vi "Get Main Menu.vi"(8 "error in":errorcluster) -> (0 "error out":errorcluster, 3 "Main Menu":T1)   [LabVIEW 2026]
doc: "Returns the ATM Main Menu as data: for each of the six function buttons the label shown beside it and the state the main state machine runs when it is pressed. Left side: Fast Cash $100, Balance Inquiry, Return Card and Terminate. Right side: Deposit, Withdraw, Fast Cash $50. To change a label or to move an item to another button, edit the Main Menu constant; the main state machine needs no change for that. An item with a NEW action also needs a new item in ATM States.ctl and a case for it in the main state machine - an action without a case of its own runs the \"None\", Default case and does nothing.\n\nError behaviour: error in is passed to error out unchanged; the menu is returned in every case."
uses:
  Controls/ATM Menu.ctl
  Controls/ATM Menu Side.ctl
  Controls/ATM Menu Item.ctl
  Controls/ATM States.ctl
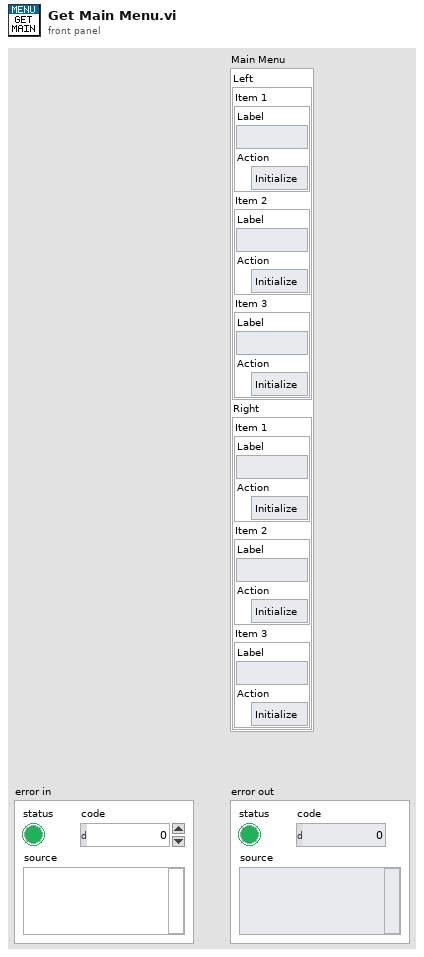
[diagram p1: front panel]
types:
  T1 = typedef "ATM Menu.ctl" = cluster{"Left":T2, "Right":T2}
  T2 = typedef "ATM Menu Side.ctl" = cluster{"Item 1":T3, "Item 2":T3, "Item 3":T3}
  T3 = typedef "ATM Menu Item.ctl" = cluster{"Label":string, "Action":T4}
  T4 = typedef "ATM States.ctl" = enum16{"Initialize", "Wait for Event", "Card Inserted", "Process Input", "Verify Account", "Show Main Menu", "Deposit Prompt", "Withdraw Prompt", "Deposit", "Withdraw", "Fast Cash", "Balance Inquiry", "None", "Terminate Session", "Exit", "Fast Cash $100"}
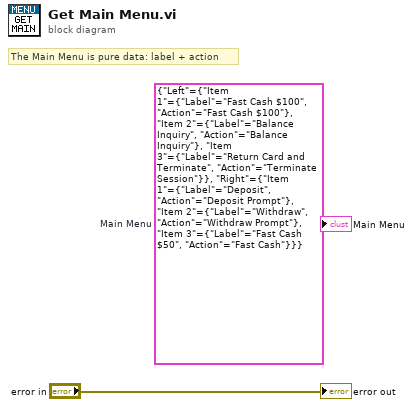
[diagram p0: block diagram]
diagram:
  w2 = T1 {"Left"={"Item 1"={"Label"="Fast Cash $100", "Action"=enum."Fast Cash $100"}, "Item 2"={"Label"="Balance Inquiry", "Action"=enum."Balance Inquiry"}, "Item 3"={"Label"="Return Card and Terminate", "Action"=enum."Terminate Session"}}, "Right"={"Item 1"={"Label"="Deposit", "Action"=enum."Deposit Prompt"}, "Item 2"={"Label"="Withdraw", "Action"=enum."Withdraw Prompt"}, "Item 3"={"Label"="Fast Cash $50", "Action"=enum."Fast Cash"}}}  # Main Menu
  # "The Main Menu is pure data: label + action"
  "Main Menu" <- w2
  "error out" <- "error in"
